vi "XIS Get Integration Times.vi"(8 "error in (no error)":errorcluster, 10 "count":i32=8, 11 "timesArray":dbl[](array[numeric])) -> (0 "error out":errorcluster, 1 "function return":i32, 2 "count out":i32, 3 "timesArray out":dbl[](array[numeric]))   [LabVIEW 2025, in "VarexWrapper.lvlib"]
doc: "VAREX_API int XIS_GetIntegrationTimes(double* timesArray, int* count);"
uses:
  VarexWrapper.lvlib
  VarexWrapper.dll
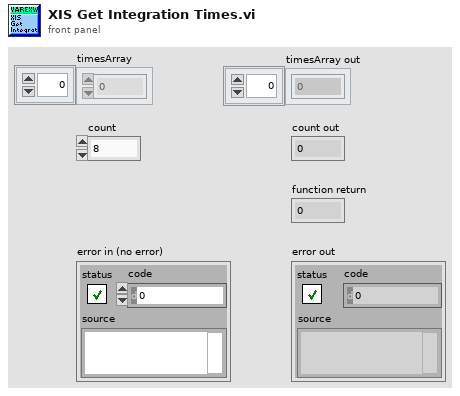
[diagram p1: front panel]
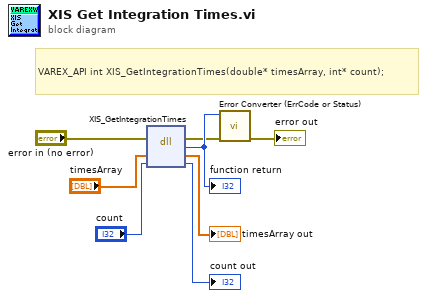
[diagram p0: block diagram]
diagram:
  # "VAREX_API int XIS_GetIntegrationTimes(double* timesArray, int* count);"
  n1 = dll-call lib="C:/Users/AriNutpam User/Documents/GitHub/The-Oracle/Image Acquisition/Child Classes/VarexImager/VarexWrapperLvLib/VarexWrapper.*" fn="XIS_GetIntegrationTimes"(error in="error in (no error)", "timesArray"="timesArray", "count"="count") -> (error out=w2:errorcluster, "return type"=w8:i32, "timesArray"=→"timesArray out":dbl[], "count"=→"count out":i32)  [unwired: 2 in, 1 out]
  "function return" <- w8
  n2 = call "Error Converter (ErrCode or Status).vi"("error in (no error)"=w2, "error code"=w8) -> ("error out"=→"error out":errorcluster)  [unwired: 9 in]
